vi "SubTask1.vi"   [LabVIEW 2016, in "PMR_081.lvrbt"]
uses:
  PMR_081.lvrbt
  <vilib>/NXT/Block Support/NXT_InputPort.ctl
  <vilib>/NXT/Block Support/NXT_OutputPort.ctl
  <vilib>/NXT/Dual Mode Library/Sensors/EV3_Color_Color.vi
  <vilib>/NXT/NXTIO Xnodes/NXTIONodeSubVIs/NXTMoveMotors.vi
  <vilib>/NXT/NXTIO Xnodes/NXTIONodeSubVIs/NXTStopMotors.vi
  <vilib>/NXT/NXTIO Xnodes/AddressXNode/NXTIOAddress.xnode
  <vilib>/NXT/Subs/LVHSConnector.ctl
  <vilib>/NXT/NXTIO Xnodes/NXTIOXNode/NXTIO.xnode
  <vilib>/NXT/LegoClasses/BrickReference/BrickReference.lvclass
types:
  T1 = typedef "NXT_InputPort.ctl" = u32
  T2 = typedef "ColorSensorColors.ctl" = enum16{"No Color", "Black", "Blue", "Green", "Yellow", "Red", "White", "Brown"}
  T3 = typedef "NXT_OutputPort.ctl" = u8
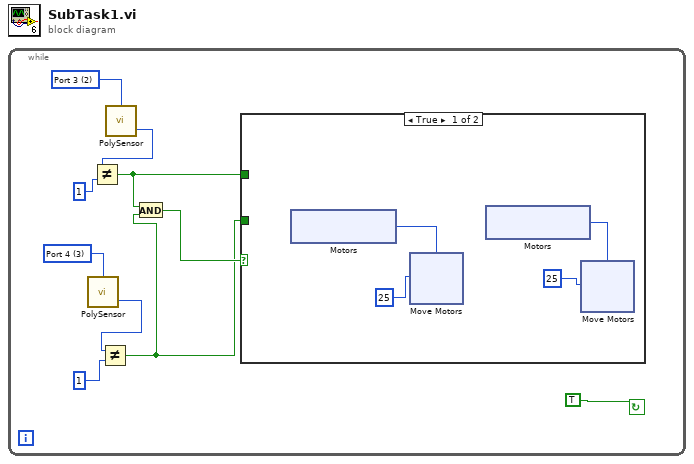
[diagram p0: block diagram]
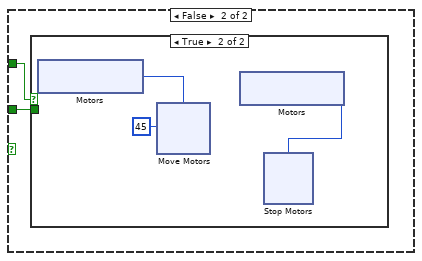
[diagram p2: hidden frame]
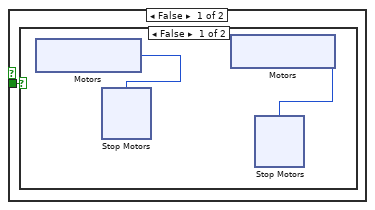
[diagram p3: hidden frame]
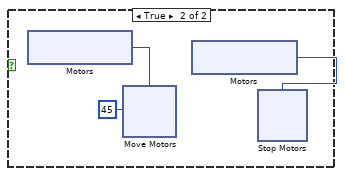
[diagram p4: hidden frame]
diagram:
  n1 = while {
    stop <- TRUE continue-if-true
    w9 = T1 3 items=["Port 1", "Port 2", "Port 3", "Port 4"] ("Port (Port 1)")
    w10 = T1 2 items=["Port 1", "Port 2", "Port 3", "Port 4"] ("Port (Port 1)")
    n2 = call-poly <vilib>:"PolySensor.vi"("Port (Port 1)"=w9) -> ("Detected Color"=w4:T2)  [unwired: 2 in, 1 out]
    n3 = Not Equal?(x=w4, y=1) -> (x != y?=w1:bool)
    n4 = call-poly <vilib>:"PolySensor.vi"("Port (Port 1)"=w10) -> ("Detected Color"=w6:T2)  [unwired: 2 in, 1 out]
    n5 = Not Equal?(x=w6, y=1) -> (x != y?=w2:bool)
    n6 = And(x=w2, y=w1) -> (x .and. y?=w8:bool)
    n7 = case shown="True" w8 {
      tunnel: w2 -> [_ w32]
      tunnel: w1 -> [_ w31]
      frame True {
        n8 = xnode "Motors"() -> ("Motor"=w12:T3)
        n9 = xnode "Move Motors"("Power/Speed 1"=i8 25, "Motors"=w12) -> ()  [unwired: 1 in, 1 out]
        n10 = xnode "Motors"() -> ("Motor"=w11:T3)
        n11 = xnode "Move Motors"("Power/Speed 1"=i8 25, "Motors"=w11) -> ()  [unwired: 1 in, 1 out]
      }
      frame False {
        n12 = case shown="True" w32 {
          tunnel: w31 -> [w33 _]
          frame False {
            n13 = case shown="False" w33 {
              frame False {
                n14 = xnode "Motors"() -> ("Motor"=w35:T3)
                n15 = xnode "Stop Motors"("Motors"=w35) -> ()  [unwired: 1 in, 1 out]
                n16 = xnode "Motors"() -> ("Motor"=w34:T3)
                n17 = xnode "Stop Motors"("Motors"=w34) -> ()  [unwired: 1 in, 1 out]
              }
              frame True {
                n18 = xnode "Motors"() -> ("Motor"=w50:T3)
                n19 = xnode "Move Motors"("Power/Speed 1"=i8 45, "Motors"=w50) -> ()  [unwired: 1 in, 1 out]
                n20 = xnode "Motors"() -> ("Motor"=w48:T3)
                n21 = xnode "Stop Motors"("Motors"=w48) -> ()  [unwired: 1 in, 1 out]
              }
            }
          }
          frame True {
            n22 = xnode "Motors"() -> ("Motor"=w66:T3)
            n23 = xnode "Move Motors"("Power/Speed 1"=i8 45, "Motors"=w66) -> ()  [unwired: 1 in, 1 out]
            n24 = xnode "Motors"() -> ("Motor"=w65:T3)
            n25 = xnode "Stop Motors"("Motors"=w65) -> ()  [unwired: 1 in, 1 out]
          }
        }
      }
    }
  }
